vi "VIH HelpGen - HREF - Refresh Links in Description.vi"(7 "HTML Folder":path, 11 "Description in":string) -> (3 "Description out":string)   [LabVIEW 2014]
doc: "::: VI Helpeks :::\nCopyright (c) 2000-2026 Konstantin Shifershteyn. All rights reserved."
panel:
  # "<a href=\"hprj:VM - 2D Array of DBL.vi\">VM - 2D Array of DBL</a>"
  # "VI Helpeks\nCopyright (c) 2012-2026 Konstantin Shifershteyn"
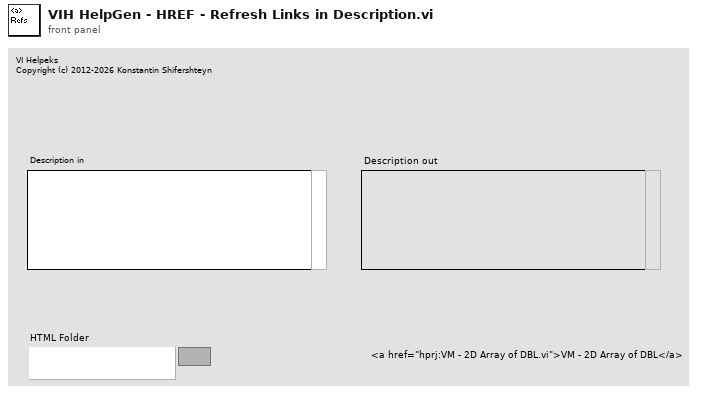
[diagram p1: front panel]
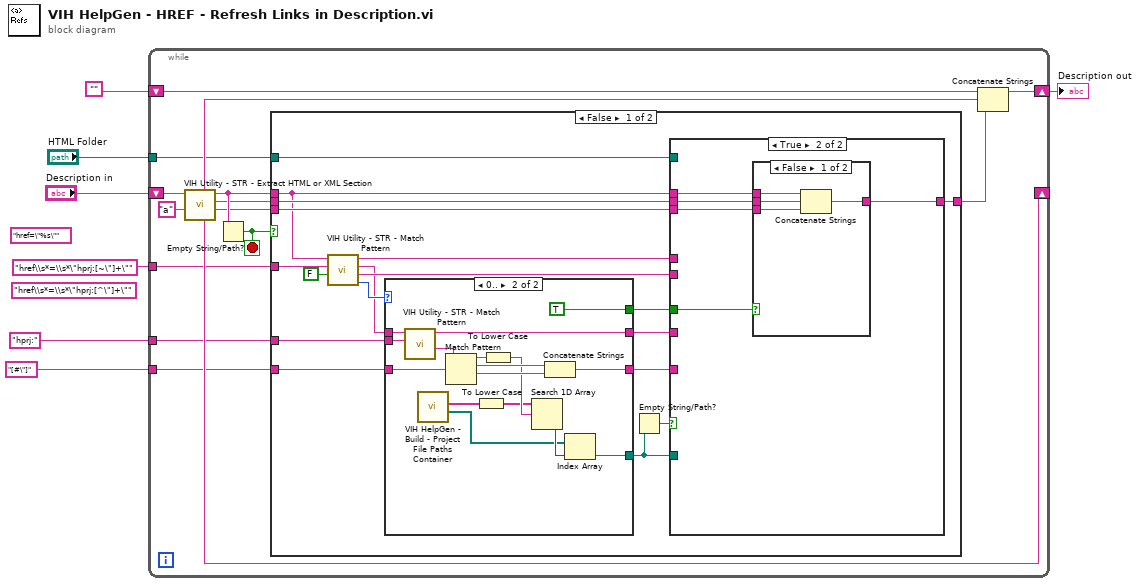
[diagram p0: block diagram]
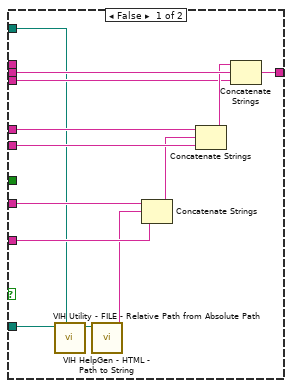
[diagram p2: hidden frame]
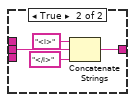
[diagram p3: hidden frame]
diagram:
  (unwired) "href\\s*=\\s*\"hprj:[^\"]+\""
  (unwired) "href=\"%s\""
  n1 = while {
    shift-right: [w20] -> _
    shift-left: "Description in" -> [w22]
    shift-right: [w17] -> w5
    shift-left: "" -> [w18]
    tunnel: "href\\s*=\\s*\"hprj:[~\"]+\"" -> [w16]
    tunnel: "hprj:" ("Regular expression") -> [w10]
    tunnel: "[#\"]" ("regular expression") -> [w9]
    tunnel: "HTML Folder" -> [w8]
    stop <- w12 stop-if-true
    n2 = call "VIH Utility - STR - Extract HTML or XML Section.vi"("Section name"="a", "HTML in"=w22) -> ("end"=w11:string, "body"=w15:string, "start"=w19:string, "after"=w20:string, "before"=w13:string)  [unwired: 5 in]
    n3 = Empty String/Path?(string/path=w19) -> (empty?=w12:bool)
    n4 = case shown="False" w12 {
      tunnel: w19 -> [w23 _]
      tunnel: w16 -> [w39 _]
      tunnel: w15 -> [w36 _]
      tunnel: [w37 _] -> w14
      tunnel: w11 -> [w35 _]
      tunnel: w10 -> [w27 _]
      tunnel: w9 -> [w26 _]
      tunnel: w8 -> [w25 _]
      frame False {
        n5 = call "VIH Utility - STR - Match Pattern.vi"("case-sensitive (F)"=FALSE, "Regular expression"=w39, "String"=w23) -> ("offset past match"=w38:i32, "after substring"=w33:string, "match substring"=w32:string, "before substring"=w34:string)  [unwired: 5 in]
        n6 = case shown="0.." w38 {
          tunnel: w32 -> [_ w76]
          tunnel: [_ w81] -> w31
          tunnel: [_ w75] -> w29
          tunnel: [_ w77] -> w28
          tunnel: w27 -> [_ w73]
          tunnel: w26 -> [_ w72]
          tunnel: [_ TRUE] -> w24
          frame ..-1 {
          }
          frame 0.. {
            n7 = call "VIH Utility - STR - Match Pattern.vi"("Regular expression"=w73, "String"=w76) -> ("after substring"=w74:string, "before substring"=w75:string)  [unwired: 6 in, 2 out]
            n8 = call "VIH HelpGen - Build - Project File Paths Container.vi"() -> ("HTML Paths"=w68:path[], "Item File Names"=w70:string[])  [unwired: 9 in, 1 out]
            n9 = Match Pattern(string=w74, regular expression=w72) -> (before substring=w80:string, match substring=w79:string, after substring=w78:string)  [unwired: 1 in, 1 out]
            n10 = To Lower Case(string=w70) -> (all lower case string=w69:string[])
            n11 = To Lower Case(string=w80) -> (all lower case string=w71:string)
            n12 = Search 1D Array(1D array=w69, element=w71) -> (index of element=w82:i32)  [unwired: 1 in]
            n13 = Concatenate Strings(w79, w78) -> (w77:string)
            n14 = Index Array(array=w68, index=w82) -> (element=w81:path)
          }
        }
        n15 = Empty String/Path?(string/path=w31) -> (empty?=w30:bool)
        n16 = case shown="True" w30 {
          tunnel: w36 -> [w51 w58]
          tunnel: [w48 w57] -> w37
          tunnel: w34 -> [w53 _]
          tunnel: w33 -> [w52 _]
          tunnel: w35 -> [w49 w54]
          tunnel: w31 -> [w46 _]
          tunnel: w29 -> [w45 _]
          tunnel: w28 -> [w44 _]
          tunnel: w25 -> [w41 _]
          tunnel: w24 -> [_ w56]
          tunnel: w23 -> [_ w55]
          frame False {
            n17 = call "VIH Utility - FILE - Relative Path from Absolute Path.vi"("base path (empty: dir of Top VI)"=w41, "Path"=w46) -> ("Rel Path out"=w47:path)  [unwired: 7 in, 2 out]
            n18 = call "VIH HelpGen - HTML - Path to String.vi"("Path"=w47) -> ("String"=w43:string)  [unwired: 10 in]
            n19 = Concatenate Strings(w45, w43, w44) -> (w42:string)
            n20 = Concatenate Strings(w53, w42, w52) -> (w50:string)
            n21 = Concatenate Strings(w50, w51, w49) -> (w48:string)
          }
          frame True {
            n22 = case shown="False" w56 {
              tunnel: w58 -> [w61 w66]
              tunnel: [w59 w63] -> w57
              tunnel: w55 -> [w62 _]
              tunnel: w54 -> [w60 _]
              frame False {
                n23 = Concatenate Strings(w62, w61, w60) -> (w59:string)
              }
              frame True {
                n24 = Concatenate Strings("<i>" ("element"), w66, "</i>" ("element")) -> (w63:string)
              }
            }
          }
        }
      }
      frame True {
      }
    }
    n25 = Concatenate Strings(w18, w13, w14) -> (w17:string)
  }
  "Description out" <- w5
